vi "VIH HelpGen - Image - Search Rect in Bounds Array.vi"(10 "Rect Bounds":cluster{"X0":i32, "Y0":i32, "X1":i32, "Y1":i32}, 11 "Rect array":T1(array[cluster])) -> (0 "Found Index":i32)   [LabVIEW 2014]
doc: "::: VI Helpeks :::\nCopyright (c) 2000-2026 Konstantin Shifershteyn. All rights reserved."
panel:
  # "VI Helpeks\nCopyright (c) 2012-2026 Konstantin Shifershteyn"
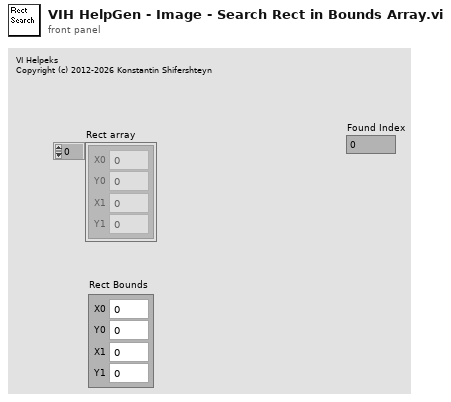
[diagram p1: front panel]
types:
  T1 = cluster{"X0":i32, "Y0":i32, "X1":i32, "Y1":i32}[]
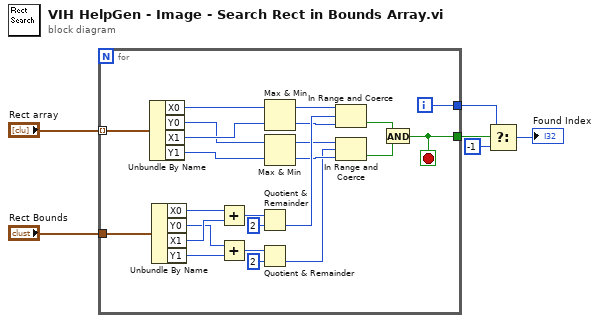
[diagram p0: block diagram]
diagram:
  n1 = for {
    tunnel: "Rect array" -> [w7] mode=indexing
    tunnel: "Rect Bounds" -> [w30]
    tunnel: [w9] -> w4
    tunnel: [w8] -> w3
    i -> [w8]
    stop <- w9 stop-if-true
    n2 = Unbundle By Name(w7) -> ("X0"=w20:i32, "Y0"=w16:i32, "X1"=w19:i32, "Y1"=w15:i32)
    n3 = Unbundle By Name(w30) -> ("X0"=w29:i32, "Y0"=w22:i32, "X1"=w28:i32, "Y1"=w23:i32)
    n4 = Add(x=w29, y=w28) -> (x+y=w27:i32)
    n5 = Add(x=w22, y=w23) -> (x+y=w24:i32)
    n6 = Quotient & Remainder(x=w27, y=2) -> (floor(x/y)=w21:i32)  [unwired: 1 out]
    n7 = Quotient & Remainder(x=w24, y=2) -> (floor(x/y)=w12:i32)  [unwired: 1 out]
    n8 = Max & Min(x=w20, y=w19) -> (max(x,y)=w18:i32, min(x,y)=w17:i32)
    n9 = Max & Min(x=w16, y=w15) -> (max(x,y)=w14:i32, min(x,y)=w13:i32)
    n10 = In Range and Coerce(upper limit=w18, x=w21, lower limit=w17) -> (In Range?=w11:bool)  [unwired: 1 out]
    n11 = In Range and Coerce(upper limit=w14, x=w12, lower limit=w13) -> (In Range?=w10:bool)  [unwired: 1 out]
    n12 = And(x=w11, y=w10) -> (x .and. y?=w9:bool)
  }
  n13 = Select(t=w3, s=w4, f=-1) -> (s? t:f=→"Found Index":i32)
